vi "Upload_test_VI_Only_Sample_v3.vi"(8 "error in":errorcluster, 11 "Initial selected EX":string[](array[string])) -> (0 "error out":errorcluster, 2 "S_Folder_path array":path[](array[path]), 3 "S_Folder array":string[](array[string]))   [LabVIEW 2018]
panel:
  out "s_path":path[](array[path])
  out "FOL# 2":i32
  out "1st 2":path[](array[path])
  out "2nd 2":path[](array[path])
  out "logical OR 4":bool
  out "logical OR 3":bool
  out "path 3":path
  out "present_s_path":path
  in  "Server selection":u16(ring) items=["Rackstation(analysis)", "Rackstation(archives)", "Rackstation(_analysis)", "QTserver(analysis)", "QTserver(backup)", "Qdserver(analysis)", "Qdserver(backup)", "QKserver(analysis)", "QKserver(backup)", "D:\\", "C:\\", "SQserver"]
  in  "All_Select":bool
  out "Folder List Array":cluster{string, bool}[](array[cluster])
  out "FOL#":i32
  out "x-1":u32
  out "SIDE":i32
  in  "Scrollbar V":i32(c297)
  out "Selected EX#":i32
  out "element":string
  in  "END":bool
  in  "All_Clear":bool
  in  "EX_IDX":i32
  out "selected folder_List":string[](array[string])
  out "Height":u32
  out "Top":i32
  out "Vertical":i32
  in  "selection":u16(ring) items=["Daicel2", "Daicel3", "Daicel_BN", "Fujishima", "Glycon", "Hitachi_N", "Kiyotani", "Kiyotani_EpPhos", "Kiyotani_HCT116", "Komoto", "Kumamoto", "Kumamoto_N2", "Mitsuzawa", "Morita_Mono", "Morita_Others", "Morita_Ox_New", "Morita_Ox_Old", "Morita_test", "Numata_N2", "Oka_1", "Oka_2", "Pan_Cancer_N2", "S49", "Sakano_00", "Sakano_01", "Sakano_02", "Sato_pep", "Seeds2025_Katahira", "Seeds2025_Maruyama", "Seeds2025_Shibata", "Seeds2025_Tada", "Seeds2025_Yasuda", "seeds2026", "Sekiya_L", "Seya", "Seya_N", "SGMO", "Shanli_mel", "Shanli_thy", "Sugar", "Suzuki_20260708", "Suzuki_2Ac", "Suzuki_2Py", "Suzuki_I", "Suzuki_Lys", "Suzuki_MLys", "Suzuki_Mlys5s", "Suzuki_MLys7s", "Suzuki_Phe", "Takahagi_2'3'RNA", "Takahagi_LaTNA", "Takahagi_LTNA", "Takahagi_LTNAn", "Takahagi_PLoop", "Takahagi_RNApeptide", "Takahagi_Zenoamino", "une", "Yamazaki"]
  out "1folder names":string[](array[string])
  out "Folder_List":string[](array[string])
  out "F_array_Link":path[](array[path])
  out "1st":path[](array[path])
  out "2nd":path[](array[path])
  out "logical OR 2":bool
  out "logical OR":bool
  out "2folder_name":string[](array[string])
  out "path":path
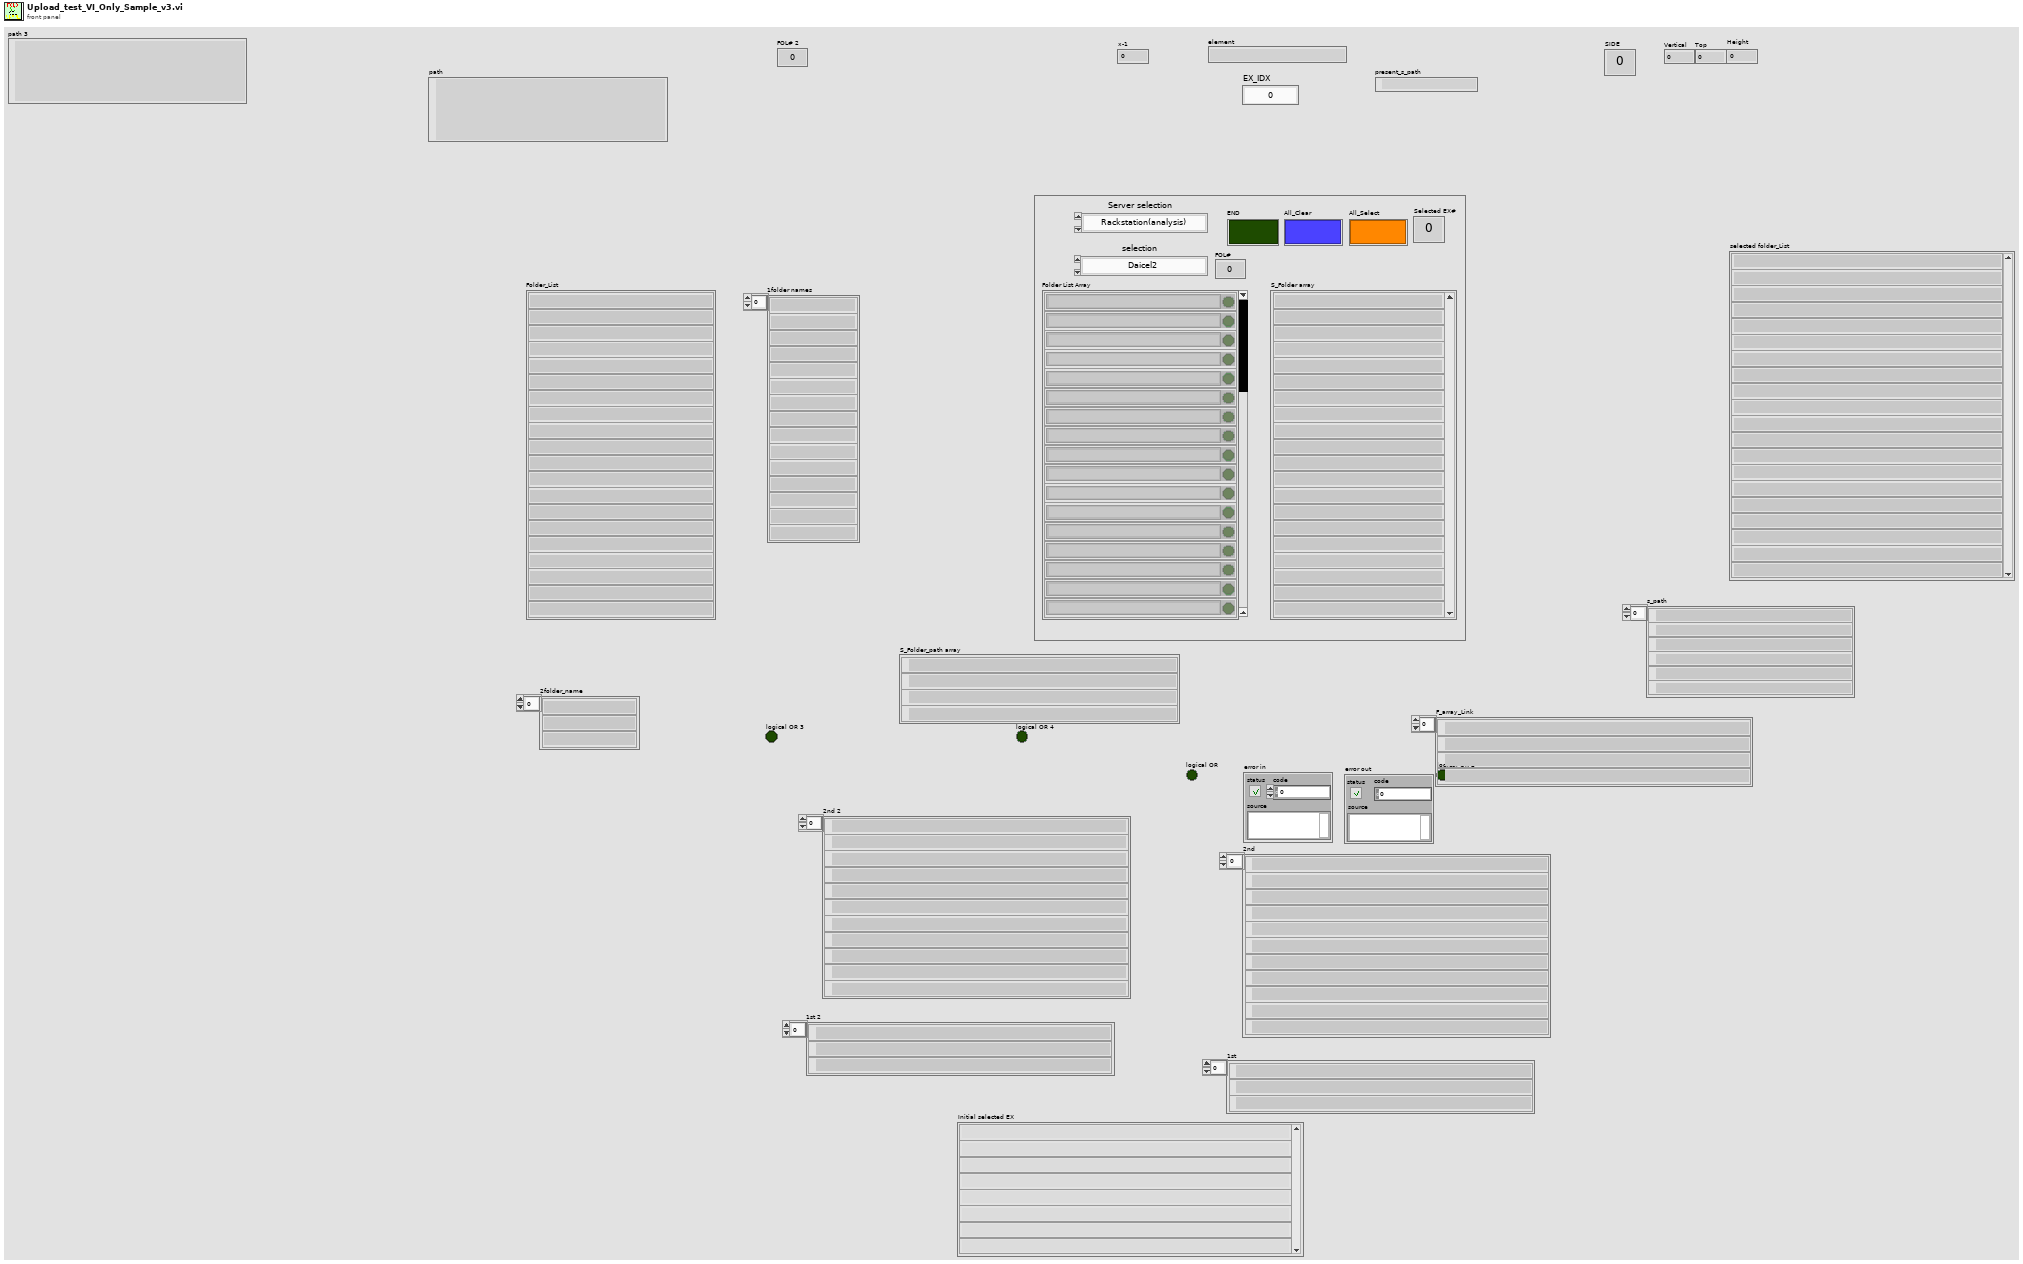
[diagram p1: front panel]
types:
  T1 = typedef "LVPoint32TypeDef.ctl" = cluster{"Horizontal":i32, "Vertical":i32}
  T2 = typedef "LVPositionTypeDef.ctl" = cluster{"Left":i32, "Top":i32}
  T3 = typedef "LVBoundsTypeDef.ctl" = cluster{"Width":u32, "Height":u32}
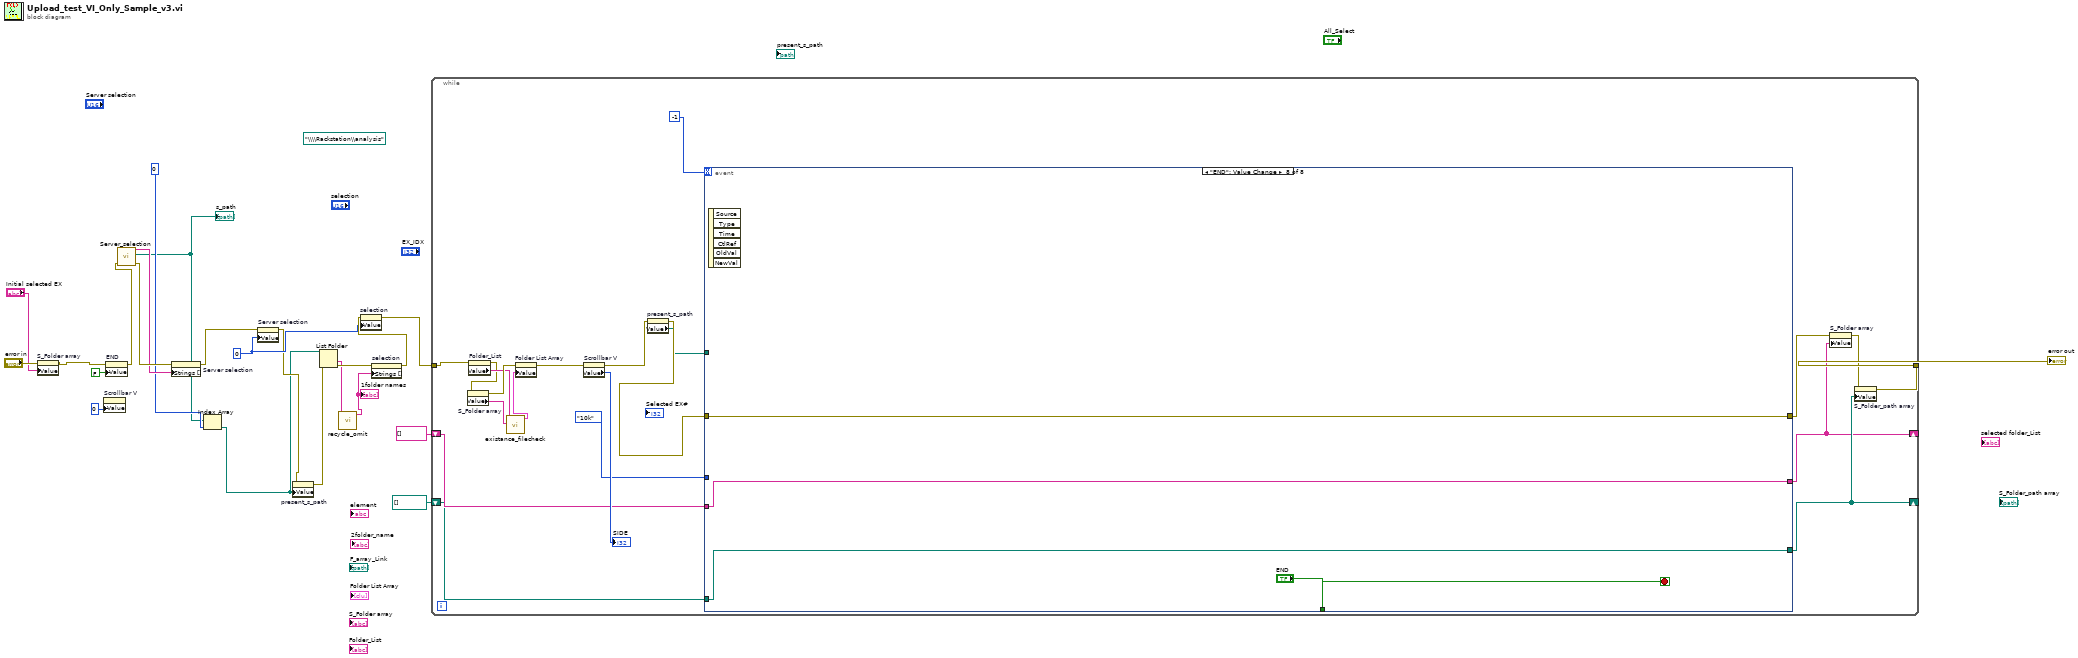
[diagram p0: block diagram]
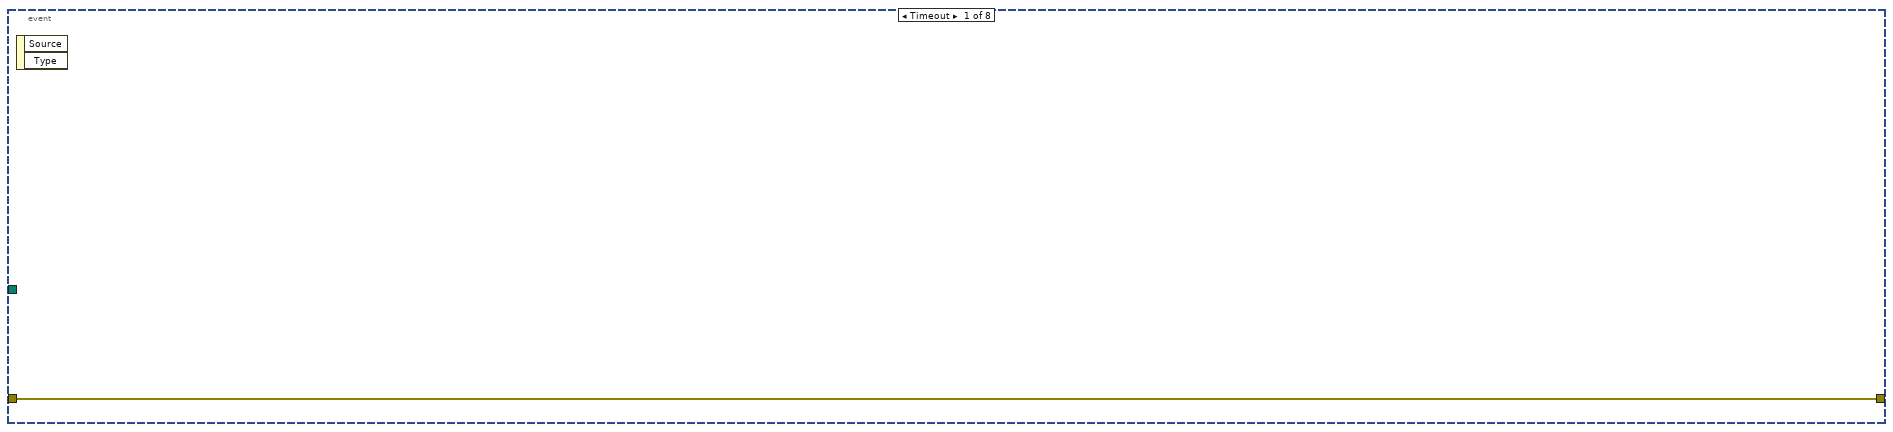
[diagram p2: hidden frame]
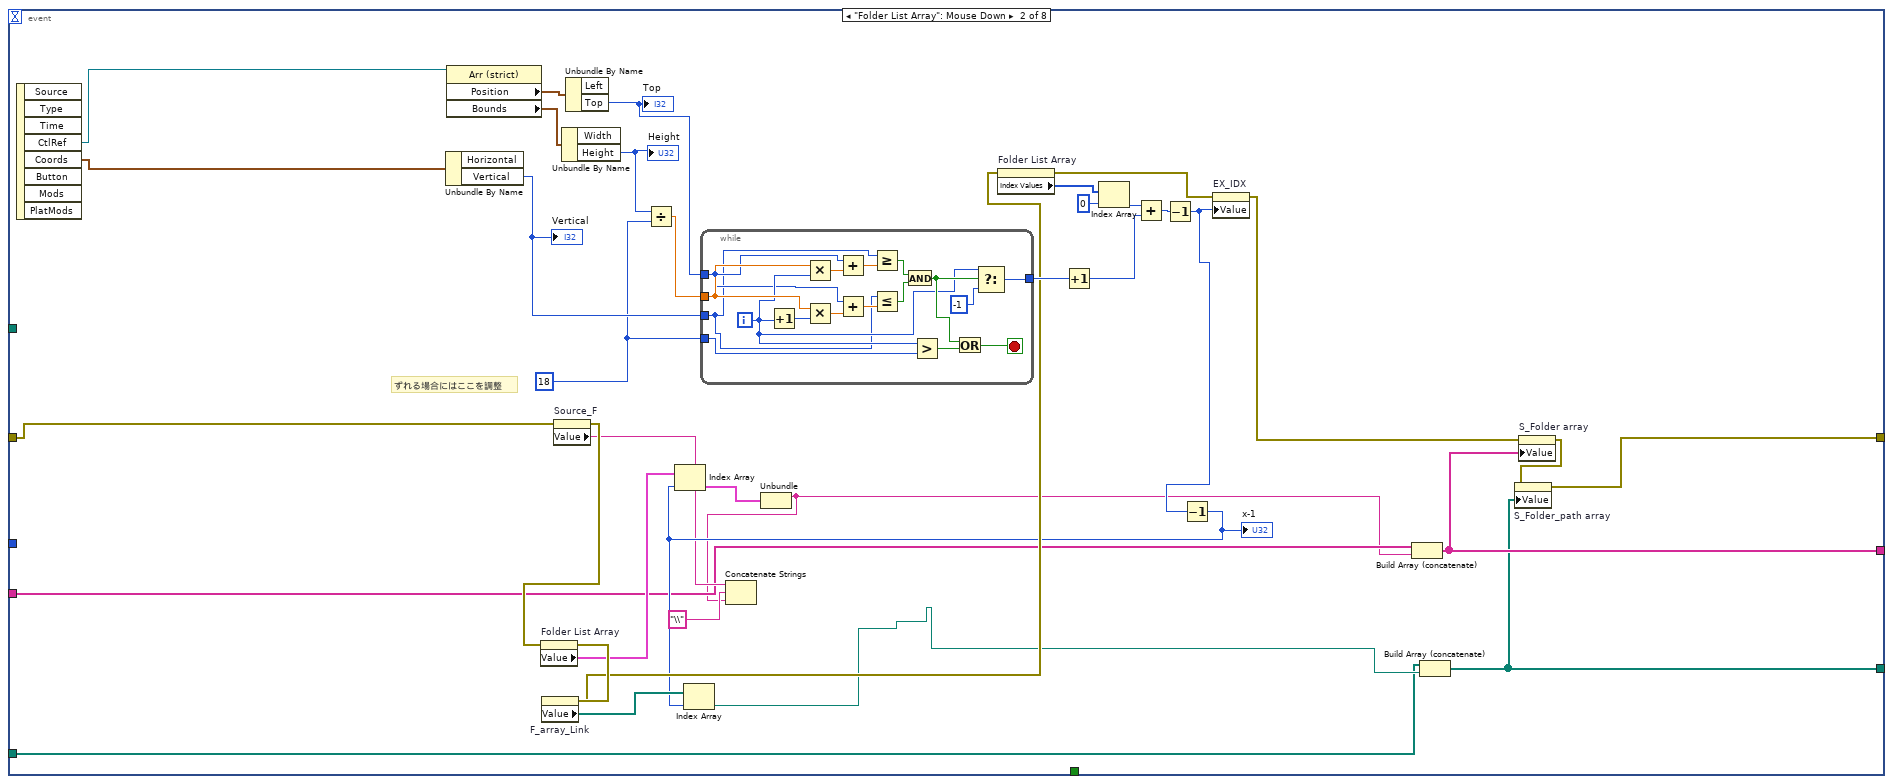
[diagram p3: hidden frame]
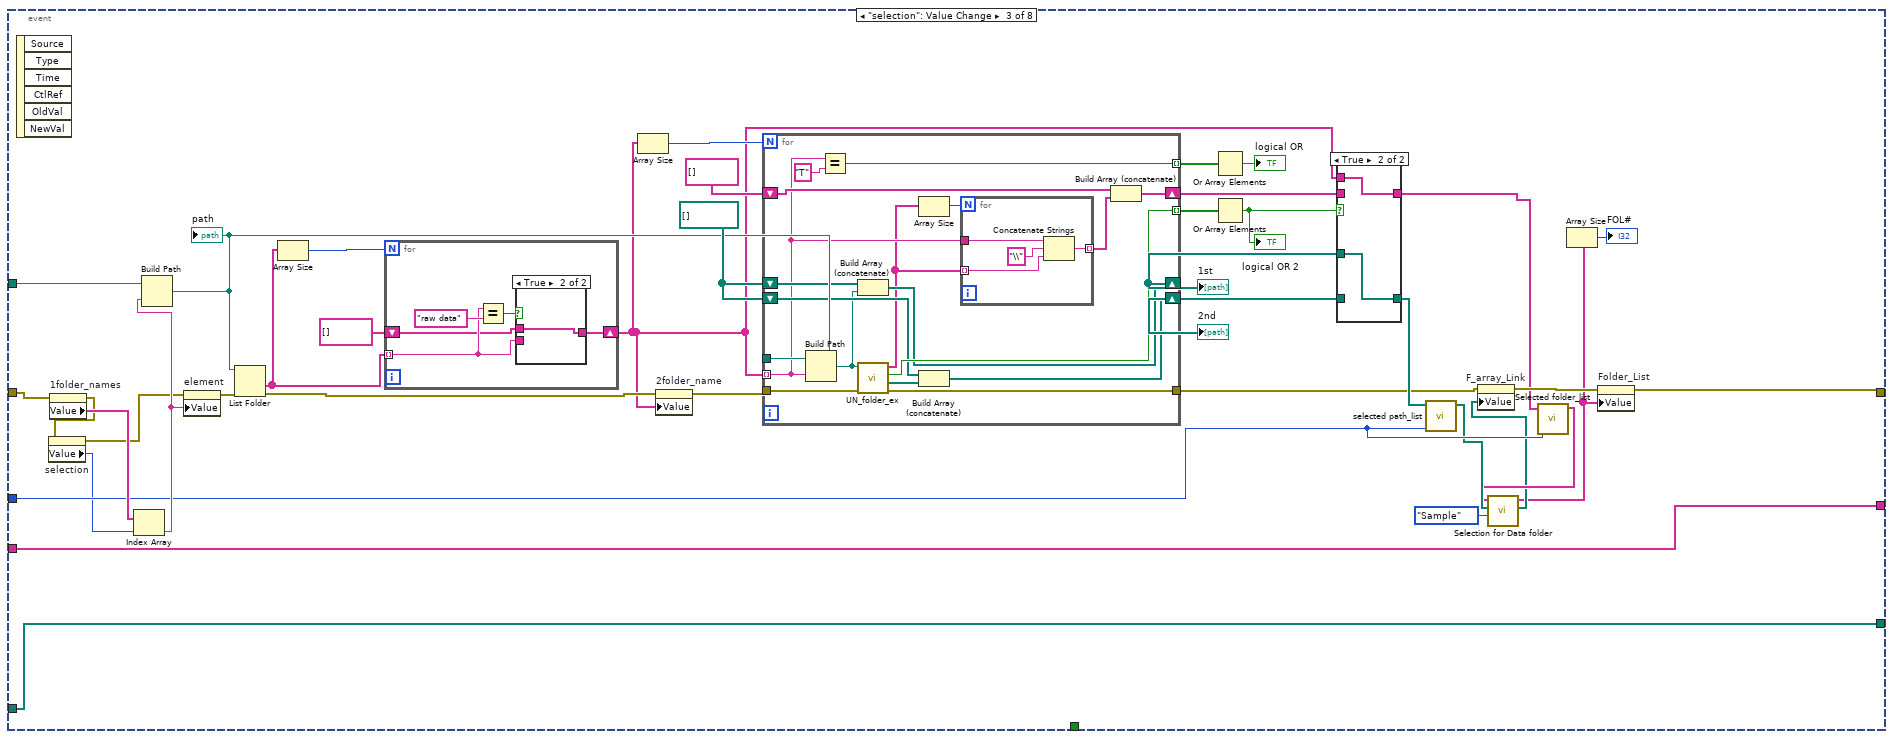
[diagram p4: hidden frame]
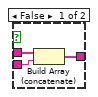
[diagram p6: hidden frame]
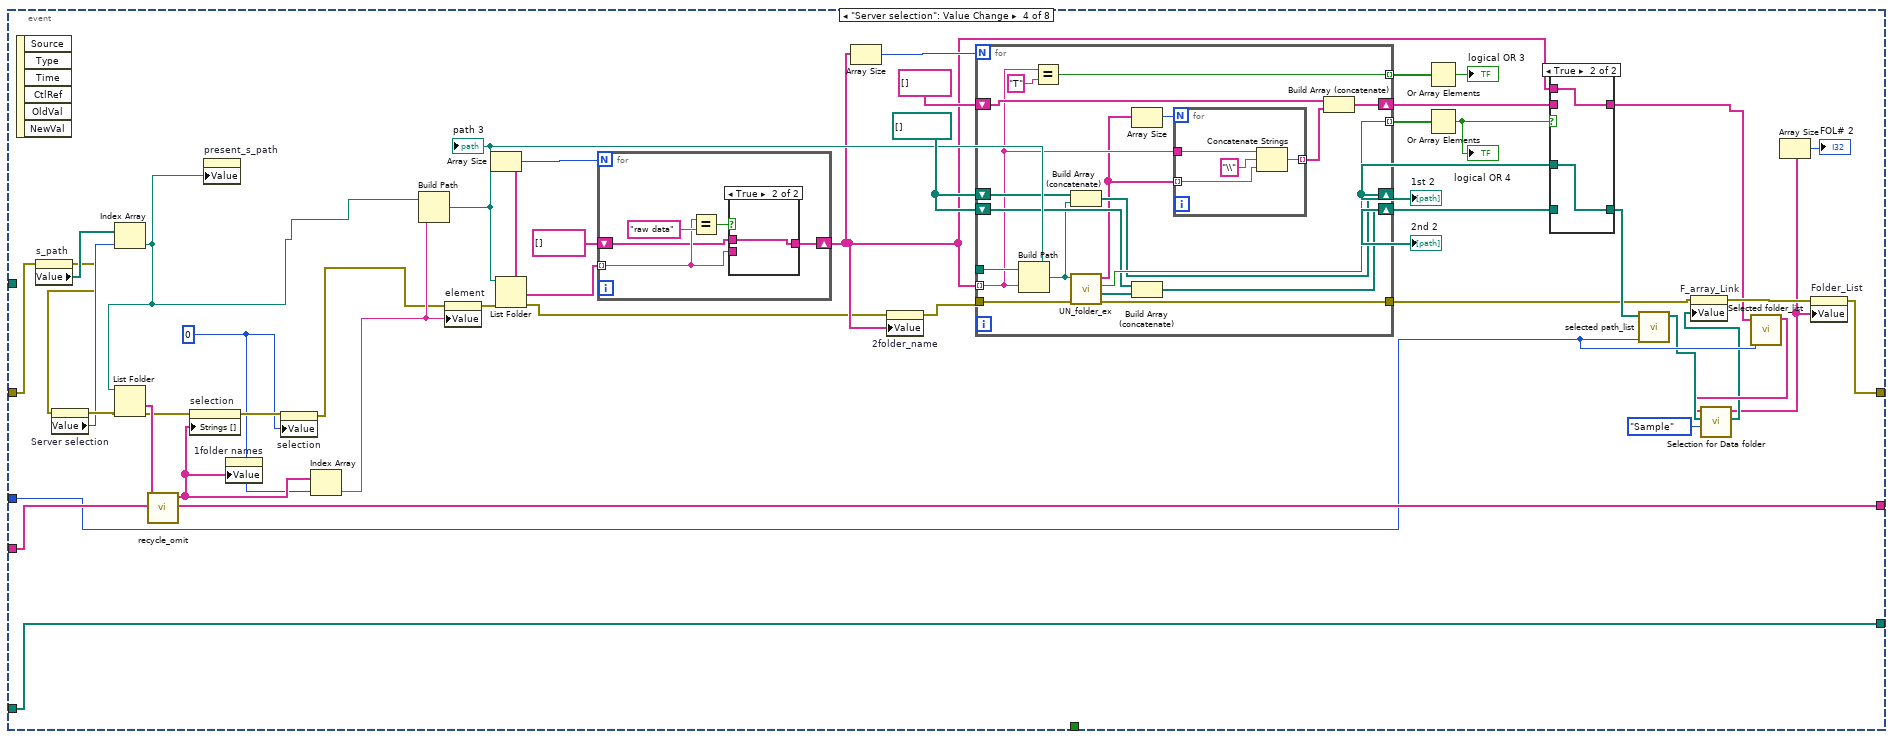
[diagram p7: hidden frame]
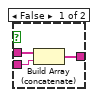
[diagram p9: hidden frame]
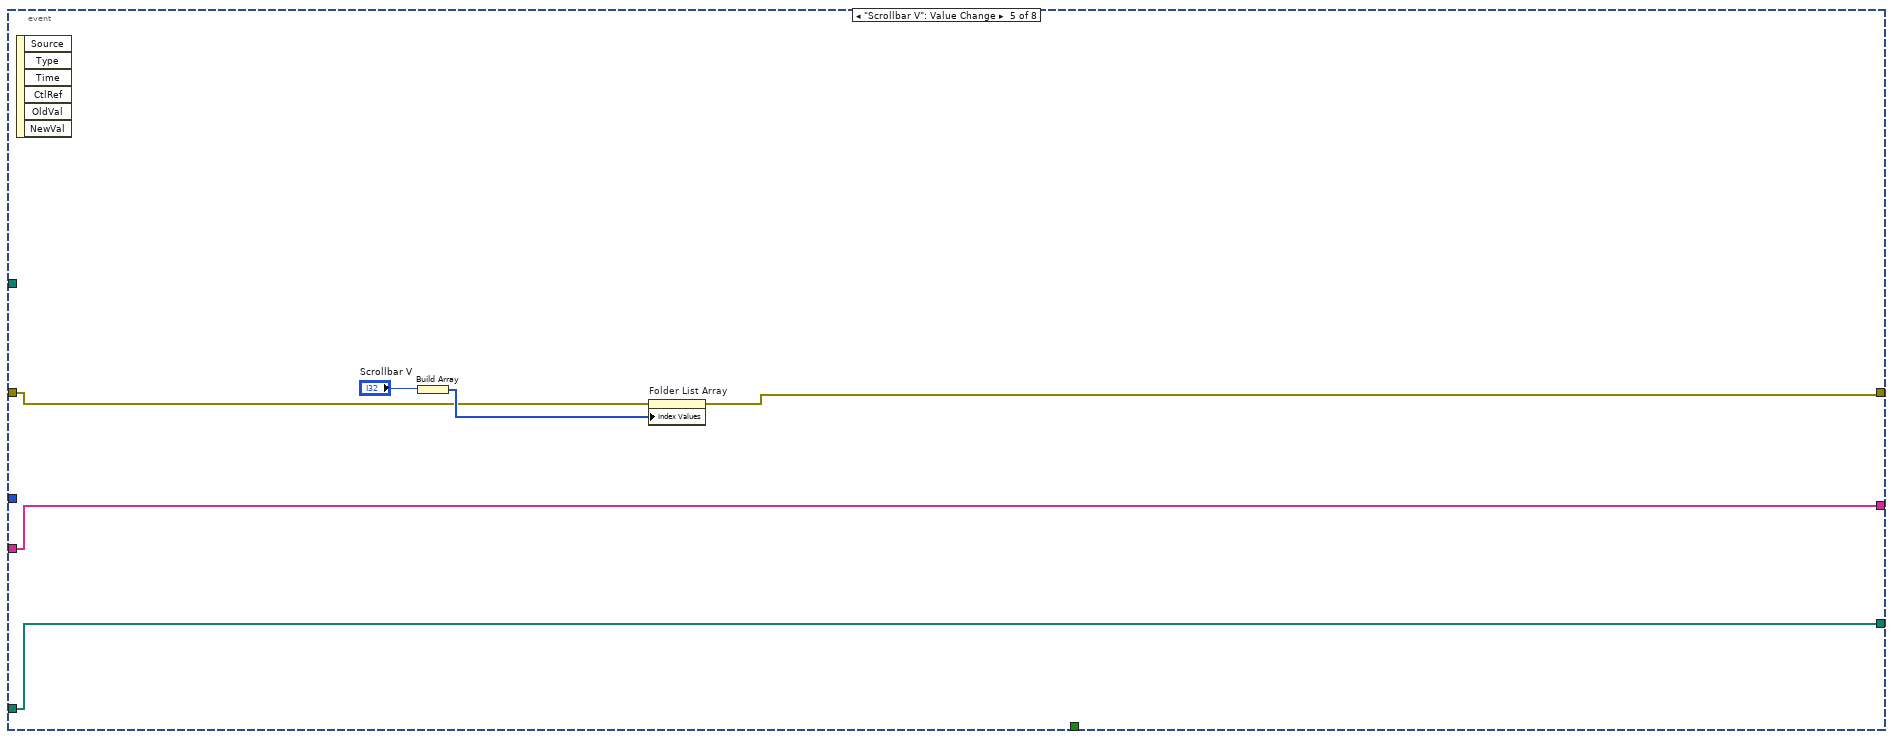
[diagram p10: hidden frame]
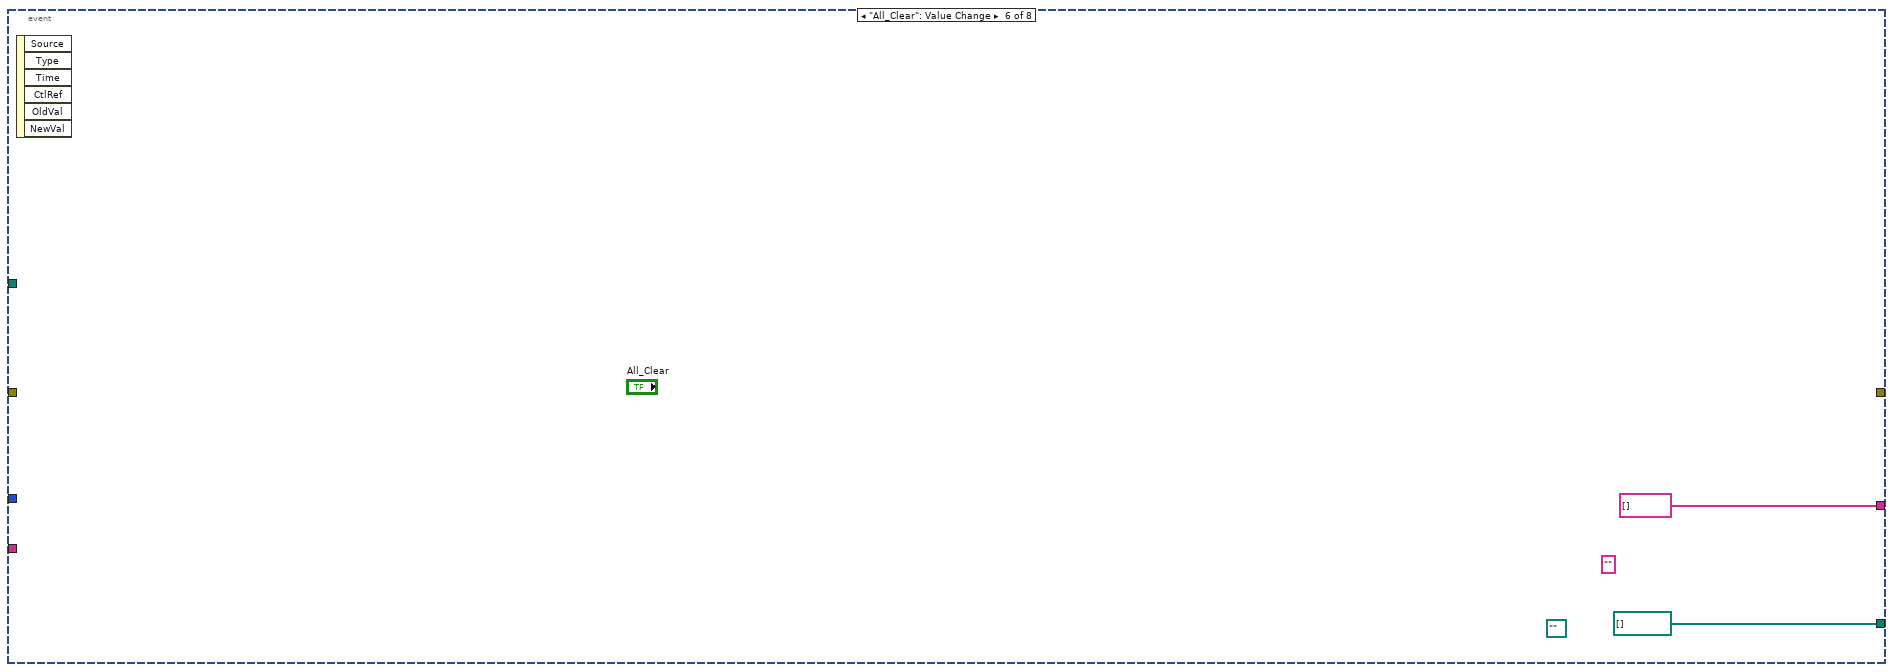
[diagram p11: hidden frame]
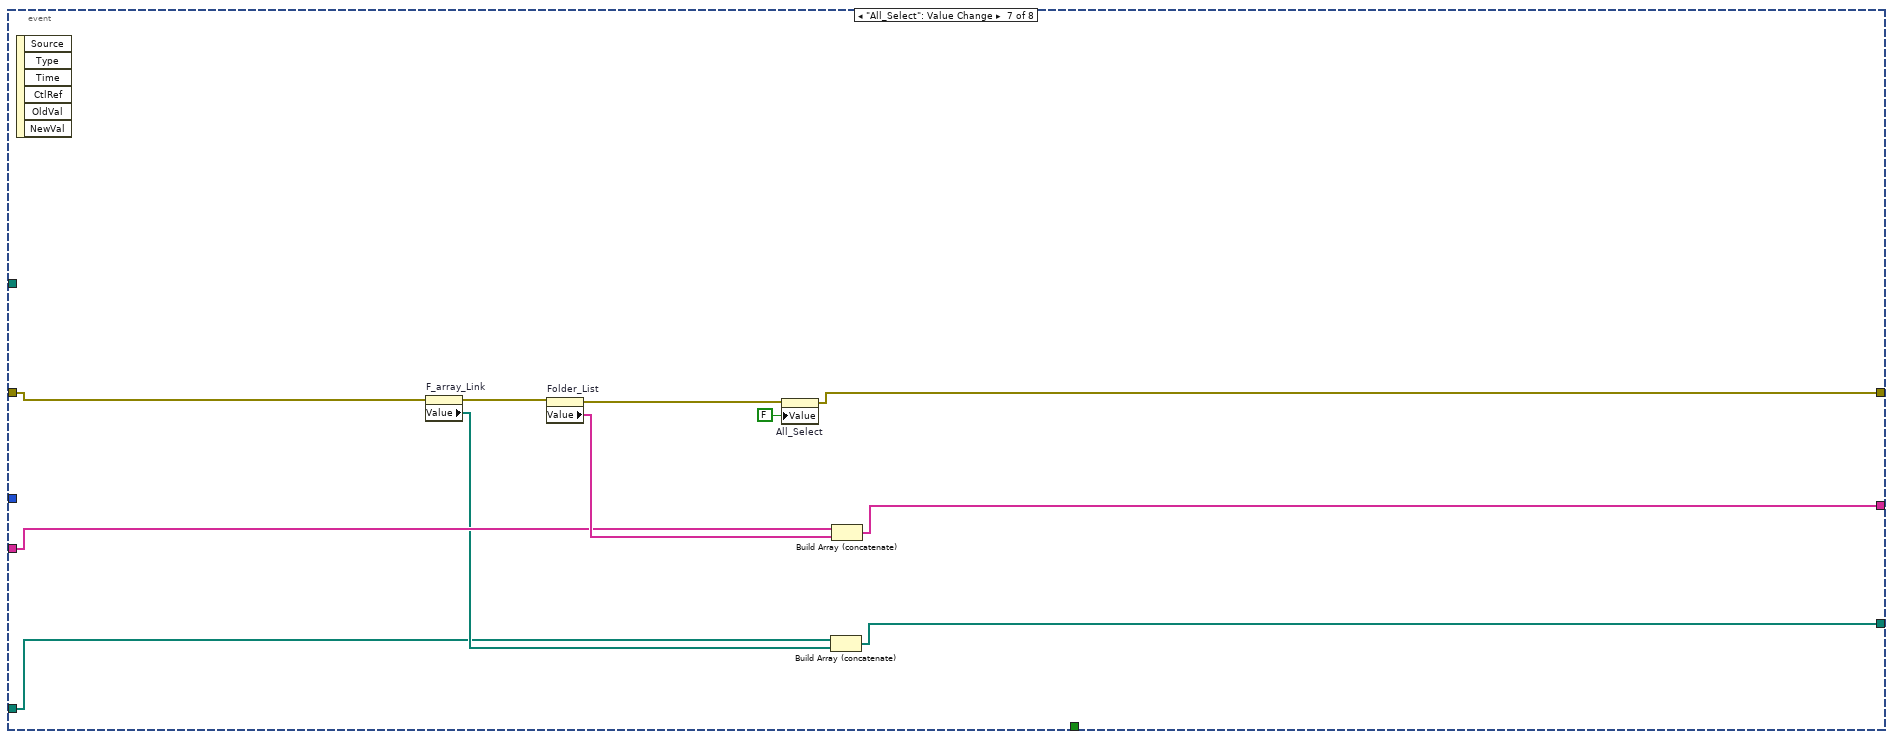
[diagram p12: hidden frame]
diagram:
  w9 = 0
  (unwired) path "\\\\Rackstation\\analysis"
  n1 = property on="S_Folder array" class="Arr (strict)"(error in="error in", "Value"="Initial selected EX") -> (error out=w16:errorcluster)  [unwired: 1 in, 1 out]
  n2 = property on="Scrollbar V" class="Scroll (strict)"("Value"=0 ("Scrollbar V")) -> ()  [unwired: 2 in, 2 out]
  n3 = property on="END" class="Bool (strict)"(error in=w16, "Value"=FALSE ("END")) -> (error out=w6:errorcluster)  [unwired: 1 in, 1 out]
  n4 = call "Server_selection.vi"("error in (no error)"=w6) -> ("error out"=w5:errorcluster, "path 2"=w2:path[], "server_name_list"=w4:string[])  [unwired: 8 in]
  "s_path" <- w2
  n5 = property on="Server selection" class="Ring (strict)"(error in=w5, "Strings []"=w4) -> (error out=w12:errorcluster)  [unwired: 1 in, 1 out]
  n6 = Index Array(array=w2, index=0) -> (element=w1:path)
  n7 = property on="Server selection" class="Ring (strict)"(error in=w12, "Value"=w9) -> (error out=w8:errorcluster)  [unwired: 1 in, 1 out]
  n8 = property on="present_s_path" class="Path"(error in=w8, "Value"=w1) -> (error out=w7:errorcluster)  [unwired: 1 in, 1 out]
  n9 = List Folder(path=w1, error in=w7) -> (folder names=w20:string[], error out=w23:errorcluster)  [unwired: 2 in, 2 out]
  n10 = call "recycle_omit.vi"("1folder names"=w20) -> ("Array"=w18:string[])  [unwired: 10 in]
  "1folder names" <- w18
  n11 = property on="selection" class="Ring (strict)"(error in=w23, "Strings []"=w18) -> (error out=w11:errorcluster)  [unwired: 1 in, 1 out]
  n12 = property on="selection" class="Ring (strict)"(error in=w11, "Value"=w9) -> (error out=w10:errorcluster)  [unwired: 1 in, 1 out]
  n13 = while {
    tunnel: w10 -> [w36]
    tunnel: [w27] -> w22
    shift-right: [w30] -> _
    shift-left: string[] [] -> [w33]
    shift-right: [w31] -> _
    shift-left: path[] [] -> [w32]
    stop <- w43 stop-if-true
    n14 = property on="Folder_List" class="Arr (strict)"(error in=w36) -> (error out=w35:errorcluster, "Value"=w37:string[])  [unwired: 1 in, 1 out]
    n15 = property on="S_Folder array" class="Arr (strict)"(error in=w35) -> (error out=w39:errorcluster, "Value"=w40:string[])  [unwired: 1 in, 1 out]
    n16 = call "existance_filecheck.vi"("selected EX"=w40, "folder names"=w37) -> ("Array 3"=w38:cluster{string, bool}[])  [unwired: 8 in, 1 out]
    n17 = property on="Folder List Array" class="Arr (strict)"(error in=w39, "Value"=w38) -> (error out=w34:errorcluster)  [unwired: 1 in, 1 out]
    n18 = property on="Scrollbar V" class="Scroll (strict)"(error in=w34) -> (error out=w26:errorcluster, "Value"=→"SIDE":i32)  [unwired: 1 in, 1 out]
    n19 = property on="present_s_path" class="Path"(error in=w26) -> (error out=w25:errorcluster, "Value"=w24:path)  [unwired: 1 in, 1 out]
    n20 = event shown="[7] \"END\": Value Change" {
      selector: _ -> [_ _ _ _ _ _ _ _]
      dyn-events: _ -> [_ _ _ _ _ _ _ _]
      timeout: -1 -> [_ _ _ _ _ _ _ _]
      tunnel: w25 -> [w45 w57 w124 w174 w257 _ w270 w274]
      tunnel: [w45 w46 w104 w207 w256 _ w267 w274] -> w29
      tunnel: w24 -> [_ _ w122 _ _ _ _ _]
      tunnel: [_ _ _ _ _ _ _ "END"] -> w43
      tunnel: enum16{"10k", "100k"}."10k" ("SHz_selection") -> [_ _ w113 w208 _ _ _ _]
      tunnel: [_ w53 w103 w216 w254 string[] [] ("Value") w266 w273] -> w30
      tunnel: w33 -> [_ w54 w103 w216 w254 _ w264 w273]
      tunnel: [_ w48 w102 w217 w253 path[] [] ("Value") w263 w272] -> w31
      tunnel: w32 -> [_ w49 w102 w217 w253 _ w261 w272]
      event Timeout {
        n21 = event-data() -> ()  [unwired: 1 in, 2 out]
      }
      event "Folder List Array": Mouse Down {
        w61 = 18 ("f")
        # "ずれる場合にはここを調整"
        n22 = event-data() -> ("CtlRef"=w59:refnum<vi>, "Coords"=w58:T1)  [unwired: 1 in, 6 out]
        n23 = Unbundle By Name(w58) -> ("Vertical"=w78:i32)  [unwired: 1 out]
        "Vertical" <- w78
        n24 = property class="Arr (strict)"(reference=w59) -> ("Position"=w80:T2, "Bounds"=w79:T3)  [unwired: 1 in, 2 out]
        n25 = property on="Source_F" class="Str"(error in=w57) -> (error out=w65:errorcluster, "Value"=w64:string)  [unwired: 1 in, 1 out]
        n26 = property on="Folder List Array" class="Arr (strict)"(error in=w65) -> (error out=w69:errorcluster, "Value"=w56:cluster{string, bool}[])  [unwired: 1 in, 1 out]
        n27 = property on="F_array_Link" class="Arr (strict)"(error in=w69) -> (error out=w68:errorcluster, "Value"=w67:path[])  [unwired: 1 in, 1 out]
        n28 = Unbundle By Name(w79) -> ("Height"=w77:u32)  [unwired: 1 out]
        "Height" <- w77
        n29 = Unbundle By Name(w80) -> ("Top"=w75:i32)  [unwired: 1 out]
        "Top" <- w75
        n30 = Divide(x=w77, y=w61) -> (x/y=w76:dbl)
        n31 = while {
          tunnel: w78 -> [w82]
          tunnel: w76 -> [w88]
          tunnel: w75 -> [w84]
          tunnel: [w93] -> w71
          tunnel: w61 -> [w83]
          i -> [w87]
          stop <- w91 stop-if-true
          n32 = Increment(x=w87) -> (x+1=w98:i32)
          n33 = Multiply(x=w88, y=w87) -> (x*y=w85:dbl)
          n34 = Multiply(x=w88, y=w98) -> (x*y=w96:dbl)
          n35 = Add(x=w84, y=w85) -> (x+y=w86:dbl)
          n36 = Add(x=w84, y=w96) -> (x+y=w97:dbl)
          n37 = Greater Or Equal?(x=w82, y=w86) -> (x >= y?=w95:bool)
          n38 = Less Or Equal?(x=w82, y=w97) -> (x <= y?=w94:bool)
          n39 = And(x=w95, y=w94) -> (x .and. y?=w90:bool)
          n40 = Greater?(x=w87, y=w83) -> (0:w89:bool)
          n41 = Or(x=w90, y=w89) -> (x .or. y?=w91:bool)
          n42 = Select(t=w87, s=w90, f=-1) -> (s? t:f=w93:i32)
        }
        n43 = property on="Folder List Array" class="Arr (strict)"(error in=w68) -> (error out=w70:errorcluster, "Index Values"=w81:u32[])  [unwired: 1 in, 1 out]
        n44 = Increment(x=w71) -> (x+1=w74:i32)
        n45 = Index Array(array=w81, index=0 ("指標")) -> (element=w72:u32)
        n46 = Add(x=w72, y=w74) -> (x+y=w73:u32)
        n47 = Decrement(x=w73) -> (x-1=w63:u32)
        n48 = Decrement(x=w63) -> (x-1=w66:u32)
        "x-1" <- w66
        n49 = Index Array(array=w56, index=w66) -> (element=w55:cluster{string, bool})
        n50 = Index Array(array=w67, index=w66) -> (element=w50:path)
        n51 = Unbundle(w55) -> (w51:string)  [unwired: 1 out]
        n52 = Concatenate Strings(w64, "\\" ("string"), w51) -> ()  [unwired: 1 out]
        n53 = property on="EX_IDX" class="DigNum (strict)"(error in=w70, "Value"=w63) -> (error out=w52:errorcluster)  [unwired: 1 in, 1 out]
        n54 = Build Array (concatenate)(w54, w51) -> (w53:string[])
        n55 = Build Array (concatenate)(w49, w50) -> (w48:path[])
        n56 = property on="S_Folder array" class="Arr (strict)"(error in=w52, "Value"=w53) -> (error out=w47:errorcluster)  [unwired: 1 in, 1 out]
        n57 = property on="S_Folder_path array" class="Arr (strict)"(error in=w47, "Value"=w48) -> (error out=w46:errorcluster)  [unwired: 1 in, 1 out]
      }
      event "selection": Value Change {
        w126 = path[] []
        n58 = event-data() -> ()  [unwired: 1 in, 6 out]
        n59 = property on="1folder_names" class="Arr (strict)"(error in=w124) -> (error out=w100:errorcluster, "Value"=w123:string[])  [unwired: 1 in, 1 out]
        n60 = property on="selection" class="Ring (strict)"(error in=w100) -> (error out=w99:errorcluster, "Value"=w101:u16)  [unwired: 1 in, 1 out]
        n61 = Index Array(array=w123, index=w101) -> (element=w116:string)
        n62 = Build Path(base path=w122, name or relative path=w116) -> (appended path=w121:path)
        "path" <- w121
        n63 = property on="element" class="Str"(error in=w99, "Value"=w116) -> (error out=w115:errorcluster)  [unwired: 1 in, 1 out]
        n64 = List Folder(path=w121, error in=w115) -> (folder names=w132:string[], error out=w120:errorcluster)  [unwired: 2 in, 2 out]
        n65 = Array Size(array=w132) -> (size(s)=w133:i32)
        n66 = for {
          N: w133 -> [_]
          tunnel: w132 -> [w144] mode=indexing
          shift-right: [w143] -> w119
          shift-left: string[] [] -> [w142]
          n67 = Equal?(x=w144, y="raw data") -> (x = y?=w145:bool)
          n68 = case shown="True" w145 {
            tunnel: w144 -> [w149 _]
            tunnel: [w148 w150] -> w143
            tunnel: w142 -> [w147 w150]
            frame False {
              n69 = Build Array (concatenate)(w147, w149) -> (w148:string[])
            }
            frame True {
            }
          }
        }
        n70 = Array Size(array=w119) -> (size(s)=w137:i32)
        n71 = property on="2folder_name" class="Arr (strict)"(error in=w120, "Value"=w119) -> (error out=w118:errorcluster)  [unwired: 1 in, 1 out]
        n72 = for {
          N: w137 -> [_]
          tunnel: w119 -> [w153] mode=indexing
          tunnel: w118 -> [w165]
          tunnel: [w167] -> w136 mode=indexing
          tunnel: w121 -> [w166]
          tunnel: [w164] -> w105
          tunnel: [w163] -> w134 mode=indexing
          shift-right: [w161] -> w130
          shift-left: w126 -> [w160]
          shift-right: [w158] -> w129
          shift-left: w126 -> [w157]
          shift-right: [w156] -> w128
          shift-left: string[] [] -> [w155]
          n73 = Build Path(base path=w166, name or relative path=w153) -> (appended path=w159:path)
          n74 = Equal?(x=w153, y="T" ("regular expression")) -> (x = y?=w167:bool)
          n75 = Build Array (concatenate)(w157, w159) -> (w158:path[])
          n76 = call "UN_folder_ex.vi"("error in"=w165, "path"=w159) -> ("error out"=w164:errorcluster, "Array"=w162:path[], "logical OR"=w163:bool, "foldername"=w152:string[])  [unwired: 6 in]
          n77 = Array Size(array=w152) -> (size(s)=w154:i32)
          n78 = Build Array (concatenate)(w160, w162) -> (w161:path[])
          n79 = for {
            N: w154 -> [_]
            tunnel: w153 -> [w172]
            tunnel: w152 -> [w171] mode=indexing
            tunnel: [w169] -> w151 mode=indexing
            n80 = Concatenate Strings(w172, "\\" ("string"), w171) -> (w169:string)
          }
          n81 = Build Array (concatenate)(w155, w151) -> (w156:string[])
        }
        "2nd" <- w130
        "1st" <- w129
        n82 = Or Array Elements(Boolean array=w136) -> (logical OR=→"logical OR":bool)
        n83 = Or Array Elements(Boolean array=w134) -> (logical OR=w131:bool)
        "logical OR 2" <- w131
        n84 = case shown="True" w131 {
          tunnel: w130 -> [w139 _]
          tunnel: [w139 w141] -> w114
          tunnel: w129 -> [_ w141]
          tunnel: w119 -> [_ w140]
          tunnel: w128 -> [w138 _]
          tunnel: [w138 w140] -> w112
          frame False {
          }
          frame True {
          }
        }
        n85 = call "selected path_list.vi"("selection"=w113, "F_array_Link"=w114) -> ("Selected F_array_Link"=w109:path[])  [unwired: 9 in]
        n86 = call "Selected folder_list.vi"("selection"=w113, "Folder_List"=w112) -> ("selected Folder List"=w108:string[])  [unwired: 9 in]
        n87 = call "Selection for Data folder.vi"("Select"=enum16{"Sample", "Blank"}."Sample", "F_array_Link"=w109, "Folder_List"=w108) -> ("S_F_array_Link"=w107:path[], "S_Folder_List"=w106:string[])  [unwired: 7 in]
        n88 = property on="F_array_Link" class="Arr (strict)"(error in=w105, "Value"=w107) -> (error out=w117:errorcluster)  [unwired: 1 in, 1 out]
        n89 = Array Size(array=w106) -> (size(s)=→"FOL#":i32)
        n90 = property on="Folder_List" class="Arr (strict)"(error in=w117, "Value"=w106) -> (error out=w104:errorcluster)  [unwired: 1 in, 1 out]
      }
      event "Server selection": Value Change {
        w195 = path[] []
        w210 = 0
        n91 = event-data() -> ()  [unwired: 1 in, 6 out]
        n92 = property on="s_path" class="Arr (strict)"(error in=w174) -> (error out=w173:errorcluster, "Value"=w175:path[])  [unwired: 1 in, 1 out]
        n93 = property on="Server selection" class="Ring (strict)"(error in=w173) -> (error out=w214:errorcluster, "Value"=w177:u16)  [unwired: 1 in, 1 out]
        n94 = Index Array(array=w175, index=w177) -> (element=w176:path)
        n95 = List Folder(path=w176, error in=w214) -> (folder names=w215:string[], error out=w213:errorcluster)  [unwired: 2 in, 2 out]
        n96 = call "recycle_omit.vi"("1folder names"=w215) -> ("Array"=w211:string[])  [unwired: 10 in]
        n97 = property on="selection" class="Ring (strict)"(error in=w213, "Strings []"=w211) -> (error out=w212:errorcluster)  [unwired: 1 in, 1 out]
        n98 = property on="present_s_path" class="Path"("Value"=w176) -> ()  [unwired: 2 in, 2 out]
        n99 = property on="1folder names" class="Arr (strict)"("Value"=w211) -> ()  [unwired: 2 in, 2 out]
        n100 = property on="selection" class="Ring (strict)"(error in=w212, "Value"=w210) -> (error out=w178:errorcluster)  [unwired: 1 in, 1 out]
        n101 = Index Array(array=w211, index=w210) -> (element=w209:string)
        n102 = Build Path(base path=w176, name or relative path=w209) -> (appended path=w193:path)
        "path 3" <- w193
        n103 = property on="element" class="Str"(error in=w178, "Value"=w209) -> (error out=w191:errorcluster)  [unwired: 1 in, 1 out]
        n104 = List Folder(path=w193, error in=w191) -> (folder names=w201:string[], error out=w179:errorcluster)  [unwired: 2 in, 2 out]
        n105 = Array Size(array=w201) -> (size(s)=w202:i32)
        n106 = for {
          N: w202 -> [_]
          tunnel: w201 -> [w224] mode=indexing
          shift-right: [w223] -> w180
          shift-left: string[] [] -> [w222]
          n107 = Equal?(x=w224, y="raw data") -> (x = y?=w225:bool)
          n108 = case shown="True" w225 {
            tunnel: w224 -> [w229 _]
            tunnel: [w228 w230] -> w223
            tunnel: w222 -> [w227 w230]
            frame False {
              n109 = Build Array (concatenate)(w227, w229) -> (w228:string[])
            }
            frame True {
            }
          }
        }
        n110 = Array Size(array=w180) -> (size(s)=w206:i32)
        n111 = property on="2folder_name" class="Arr (strict)"(error in=w179, "Value"=w180) -> (error out=w181:errorcluster)  [unwired: 1 in, 1 out]
        n112 = for {
          N: w206 -> [_]
          tunnel: w180 -> [w233] mode=indexing
          tunnel: w181 -> [w245]
          tunnel: [w247] -> w205 mode=indexing
          tunnel: w193 -> [w246]
          tunnel: [w244] -> w182
          tunnel: [w243] -> w203 mode=indexing
          shift-right: [w241] -> w199
          shift-left: w195 -> [w240]
          shift-right: [w238] -> w198
          shift-left: w195 -> [w237]
          shift-right: [w236] -> w197
          shift-left: string[] [] -> [w235]
          n113 = Build Path(base path=w246, name or relative path=w233) -> (appended path=w239:path)
          n114 = Equal?(x=w233, y="T" ("regular expression")) -> (x = y?=w247:bool)
          n115 = Build Array (concatenate)(w237, w239) -> (w238:path[])
          n116 = call "UN_folder_ex.vi"("error in"=w245, "path"=w239) -> ("error out"=w244:errorcluster, "Array"=w242:path[], "logical OR"=w243:bool, "foldername"=w232:string[])  [unwired: 6 in]
          n117 = Array Size(array=w232) -> (size(s)=w234:i32)
          n118 = Build Array (concatenate)(w240, w242) -> (w241:path[])
          n119 = for {
            N: w234 -> [_]
            tunnel: w233 -> [w252]
            tunnel: w232 -> [w251] mode=indexing
            tunnel: [w249] -> w231 mode=indexing
            n120 = Concatenate Strings(w252, "\\" ("string"), w251) -> (w249:string)
          }
          n121 = Build Array (concatenate)(w235, w231) -> (w236:string[])
        }
        "2nd 2" <- w199
        "1st 2" <- w198
        n122 = Or Array Elements(Boolean array=w205) -> (logical OR=→"logical OR 3":bool)
        n123 = Or Array Elements(Boolean array=w203) -> (logical OR=w200:bool)
        "logical OR 4" <- w200
        n124 = case shown="True" w200 {
          tunnel: w199 -> [w219 _]
          tunnel: [w219 w221] -> w190
          tunnel: w198 -> [_ w221]
          tunnel: w180 -> [_ w220]
          tunnel: w197 -> [w218 _]
          tunnel: [w218 w220] -> w189
          frame False {
          }
          frame True {
          }
        }
        n125 = call "selected path_list.vi"("selection"=w208, "F_array_Link"=w190) -> ("Selected F_array_Link"=w186:path[])  [unwired: 9 in]
        n126 = call "Selected folder_list.vi"("selection"=w208, "Folder_List"=w189) -> ("selected Folder List"=w185:string[])  [unwired: 9 in]
        n127 = call "Selection for Data folder.vi"("Select"=enum16{"Sample", "Blank"}."Sample", "F_array_Link"=w186, "Folder_List"=w185) -> ("S_F_array_Link"=w184:path[], "S_Folder_List"=w183:string[])  [unwired: 7 in]
        n128 = property on="F_array_Link" class="Arr (strict)"(error in=w182, "Value"=w184) -> (error out=w192:errorcluster)  [unwired: 1 in, 1 out]
        n129 = Array Size(array=w183) -> (size(s)=→"FOL# 2":i32)
        n130 = property on="Folder_List" class="Arr (strict)"(error in=w192, "Value"=w183) -> (error out=w207:errorcluster)  [unwired: 1 in, 1 out]
      }
      event "Scrollbar V": Value Change {
        n131 = event-data() -> ()  [unwired: 1 in, 6 out]
        n132 = Build Array("Scrollbar V") -> (w258:i32[])
        n133 = property on="Folder List Array" class="Arr (strict)"(error in=w257, "Index Values"=w258) -> (error out=w256:errorcluster)  [unwired: 1 in, 1 out]
      }
      event "All_Clear": Value Change {
        (unwired) ""
        (unwired) path ""
        n134 = event-data() -> ()  [unwired: 1 in, 6 out]
      }
      event "All_Select": Value Change {
        n135 = event-data() -> ()  [unwired: 1 in, 6 out]
        n136 = property on="F_array_Link" class="Arr (strict)"(error in=w270) -> (error out=w269:errorcluster, "Value"=w262:path[])  [unwired: 1 in, 1 out]
        n137 = property on="Folder_List" class="Arr (strict)"(error in=w269) -> (error out=w268:errorcluster, "Value"=w265:string[])  [unwired: 1 in, 1 out]
        n138 = property on="All_Select" class="Bool (strict)"(error in=w268, "Value"=FALSE ("All_Select")) -> (error out=w267:errorcluster)  [unwired: 1 in, 1 out]
        n139 = Build Array (concatenate)(w261, w262) -> (w263:path[])
        n140 = Build Array (concatenate)(w264, w265) -> (w266:string[])
      }
      event "END": Value Change {
        n141 = event-data() -> ()  [unwired: 1 in, 6 out]
      }
    }
    n142 = property on="S_Folder array" class="Arr (strict)"(error in=w29, "Value"=w30) -> (error out=w28:errorcluster)  [unwired: 1 in, 1 out]
    n143 = property on="S_Folder_path array" class="Arr (strict)"(error in=w28, "Value"=w31) -> (error out=w27:errorcluster)  [unwired: 1 in, 1 out]
  }
  "error out" <- w22
